vi "DSS-Tests-flatten_saltwater_param.vi"(8 "error in":errorcluster, 11 "array variant":variant) -> (0 "error out":errorcluster, 3 "flat":dbl[](array[numeric]))   [LabVIEW 2020, in "DSS-Tests.lvlib"]
doc: "Converts the Array variant of RDC-saltwater-generate_perm_param_to_share into its typed array (the type constant is bound to RDC-saltwater-param.ctl) and flattens every field of every row, in order, into one 1D DBL array."
uses:
  DSS-Tests.lvlib
  Computation/RDC-saltwater-param.ctl
  Computation/RDC-Reflection_Data_Computation.lvlib
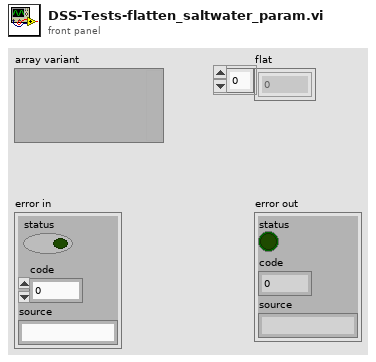
[diagram p1: front panel]
types:
  T1 = typedef "RDC-Reflection_Data_Computation.lvlib/RDC-saltwater-param.ctl" = cluster{"temp Cx10":u16, "eps s":dbl, "eps infi":dbl, "tau":dbl, "alpha":dbl, "sigma":dbl, "eps s diff":dbl, "eps infi diff":dbl, "tau diff":dbl, "alpha diff":dbl, "sigma diff":dbl}
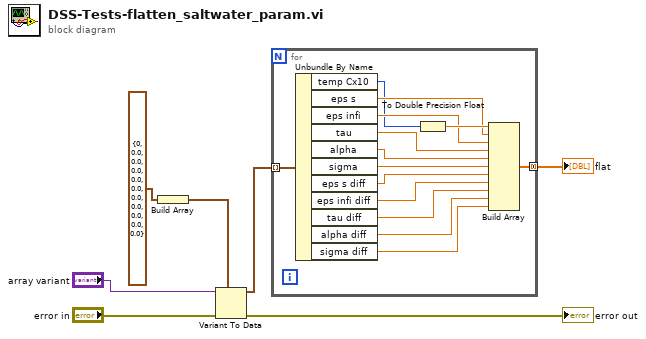
[diagram p0: block diagram]
diagram:
  n1 = Build Array(T1 {"temp Cx10"=0, "eps s"=0.0, "eps infi"=0.0, "tau"=0.0, "alpha"=0.0, "sigma"=0.0, "eps s diff"=0.0, "eps infi diff"=0.0, "tau diff"=0.0, "alpha diff"=0.0, "sigma diff"=0.0} ("water values")) -> (w4:T1[])
  n2 = Variant To Data(error in="error in", type=w4, Variant="array variant") -> (data=w5:T1[], error out=→"error out":errorcluster)
  n3 = for {
    tunnel: w5 -> [w8] mode=indexing
    tunnel: [w21] -> w7 mode=concatenating
    n4 = Unbundle By Name(w8) -> ("temp Cx10"=w9:u16, "eps s"=w10:dbl, "eps infi"=w11:dbl, "tau"=w12:dbl, "alpha"=w13:dbl, "sigma"=w14:dbl, "eps s diff"=w15:dbl, "eps infi diff"=w16:dbl, "tau diff"=w17:dbl, "alpha diff"=w18:dbl, "sigma diff"=w19:dbl)
    n5 = To Double Precision Float(number=w9) -> (double precision float=w20:dbl)
    n6 = Build Array(w20, w10, w11, w12, w13, w14, w15, w16, w17, w18, w19) -> (w21:dbl[])
  }
  "flat" <- w7
